vi "DependencyInspector.vi"(11 "Command Line Args":string[](array[string])) -> (0 "error out":errorcluster)   [LabVIEW 2020]
uses:
  UserInterface/UIManager/UIManager.lvclass
  DependencyInspection/CDependencyInspector/CDependencyInspection.lvclass
  d0761231-40dd-4f31-a9c2-62fc8e3657c5.vi/7b12b900-cc26-46dd-9914-f7ad3c9b8ec3.vi
  d0761231-40dd-4f31-a9c2-62fc8e3657c5.vi/1ae99417-134e-4b73-ab04-c2e7cd0032f4.vi
  1cd16c6c-eb87-41a4-aacc-b8daba8fd5f3.vi/7b12b900-cc26-46dd-9914-f7ad3c9b8ec3.vi
  1cd16c6c-eb87-41a4-aacc-b8daba8fd5f3.vi/1ae99417-134e-4b73-ab04-c2e7cd0032f4.vi
  <vilib>/Utility/LVClass/Get LV Class Default Value.vi
panel:
  out "Error Log":string
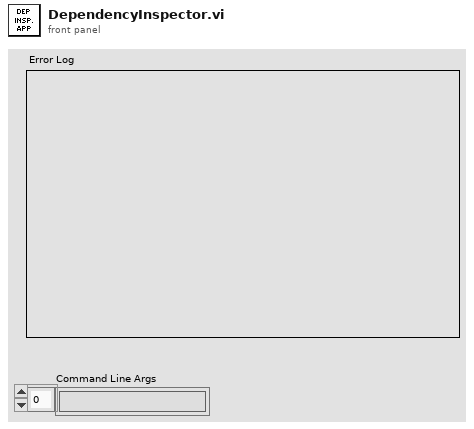
[diagram p1: front panel]
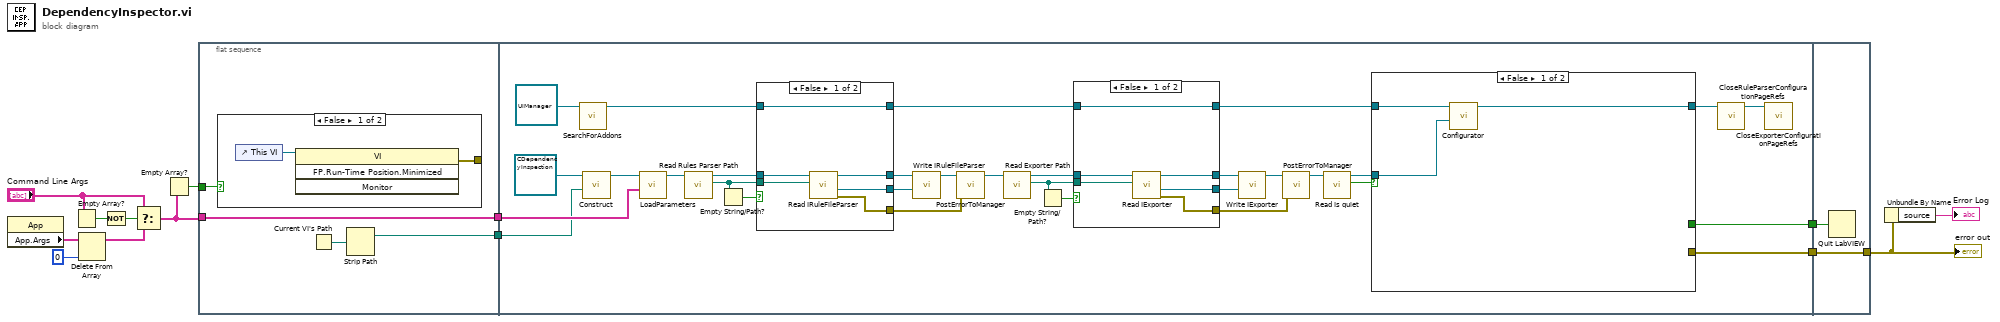
[diagram p0: block diagram]
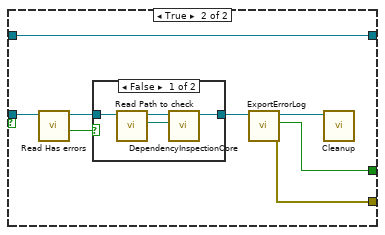
[diagram p3: hidden frame]
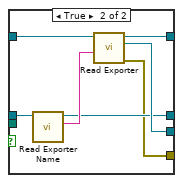
[diagram p5: hidden frame]
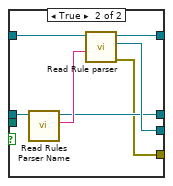
[diagram p6: hidden frame]
diagram:
  n1 = property class="App"() -> ("App.Args"=w11:string[])  [unwired: 2 in, 2 out]
  n2 = Empty Array?(array="Command Line Args") -> (empty?=w5:bool)
  n3 = Delete From Array(array=w11, index=0) -> (array with subset deleted=w4:string[])  [unwired: 1 in, 1 out]
  n4 = Not(x=w5) -> (.not. x?=w1:bool)
  n5 = Select(t="Command Line Args", s=w1, f=w4) -> (s? t:f=w3:string[])
  n6 = Empty Array?(array=w3) -> (empty?=w12:bool)
  n7 = flat-sequence {
    tunnel: w3 -> [w18]
    tunnel: [w18] -> w13
    tunnel: w12 -> [w17]
    tunnel: [w15] -> w10
    tunnel: w13 -> [w33]
    tunnel: w10 -> [w28]
    tunnel: [w32] -> w9
    tunnel: [w31] -> w8
    tunnel: [w95] -> w7
    tunnel: w9 -> [w95]
    tunnel: w8 -> [w94]
    frame #0 {
      n8 = case shown="False" w17 {
        tunnel: [w19 _] -> _
        frame False {
          n9 = control-ref of="This VI"() -> (w20:refnum<vi>)
          n10 = invoke class="VI" method="FP.Run-Time Position.Minimized"(reference=w20) -> (error out=w19:errorcluster)  [unwired: 3 in, 3 out]
        }
        frame True {
        }
      }
      n11 = Current VI's Path() -> (path=w16:path)
      n12 = Strip Path(path=w16) -> (stripped path=w15:path)  [unwired: 1 out]
    }
    frame #1 {
      n13 = call-dynamic "SearchForAddons.vi"("UIManager in"=refnum<class "UIManager.lvclass"> refnum) -> ("UIManager out"=w50:refnum<class "UIManager.lvclass">)  [unwired: 9 in, 1 out]
      n14 = call-dynamic "Construct.vi"("App path"=w28, "CDependencyInspector in"=refnum<class "CDependencyInspection.lvclass"> refnum) -> ("CDependencyInspector out"=w35:refnum<class "CDependencyInspection.lvclass">)  [unwired: 8 in, 1 out]
      n15 = call-dynamic "LoadParameters.vi"("Command line args"=w33, "CDependencyInspection in"=w35) -> ("CDependencyInspection out"=w21:refnum<class "CDependencyInspection.lvclass">)  [unwired: 8 in, 1 out]
      n16 = call-dynamic "Read Rules Parser Path.vi"("CDependencyInspection in"=w21) -> ("Path"=w41:path, "CDependencyInspection out"=w46:refnum<class "CDependencyInspection.lvclass">)  [unwired: 9 in]
      n17 = Empty String/Path?(string/path=w41) -> (empty?=w45:bool)
      n18 = case shown="False" w45 {
        tunnel: w50 -> [w86 w93]
        tunnel: [w86 w92] -> w49
        tunnel: [w84 w88] -> w43
        tunnel: w46 -> [w85 w90]
        tunnel: [w82 w89] -> w42
        tunnel: w41 -> [w83 _]
        tunnel: [w81 w87] -> w25
        frame False {
          n19 = call-dynamic "Read IRuleFileParser.vi"("Path"=w83, "CDependencyInspection in"=w85) -> ("error out"=w81:errorcluster, "IRuleFileParser"=w82:refnum<class "IRuleFileParser.lvclass">, "CDependencyInspection out"=w84:refnum<class "CDependencyInspection.lvclass">)  [unwired: 7 in]
        }
        frame True {
          n20 = call-dynamic "Read Rules Parser Name.vi"("CDependencyInspection in"=w90) -> ("Name"=w91:string, "CDependencyInspection out"=w88:refnum<class "CDependencyInspection.lvclass">)  [unwired: 9 in]
          n21 = call-dynamic "Read Rule parser.vi"("Selection"=w91, "UIManager in"=w93) -> ("error out"=w87:errorcluster, "IRuleFileParser.lvclass"=w89:refnum<class "IRuleFileParser.lvclass">, "UIManager out"=w92:refnum<class "UIManager.lvclass">)  [unwired: 5 in, 2 out]
        }
      }
      n22 = call-dynamic "Write IRuleFileParser.vi"("IRuleFileParser"=w42, "CDependencyInspection in"=w43) -> ("CDependencyInspection out"=w27:refnum<class "CDependencyInspection.lvclass">)  [unwired: 9 in]
      n23 = call-dynamic "PostErrorToManager.vi"("error in (no error)"=w25, "CDependencyInspection in"=w27) -> ("CDependencyInspection out"=w26:refnum<class "CDependencyInspection.lvclass">)  [unwired: 8 in, 1 out]
      n24 = call-dynamic "Read Exporter Path.vi"("CDependencyInspection in"=w26) -> ("Path"=w38:path, "CDependencyInspection out"=w47:refnum<class "CDependencyInspection.lvclass">)  [unwired: 9 in]
      n25 = Empty String/Path?(string/path=w38) -> (empty?=w44:bool)
      n26 = case shown="False" w44 {
        tunnel: w49 -> [w73 w80]
        tunnel: [w73 w79] -> w48
        tunnel: [w71 w75] -> w40
        tunnel: w47 -> [w72 w77]
        tunnel: [w70 w76] -> w39
        tunnel: w38 -> [w69 _]
        tunnel: [w68 w74] -> w22
        frame False {
          n27 = call-dynamic "Read IExporter.vi"("Path"=w69, "CDependencyInspection in"=w72) -> ("error out"=w68:errorcluster, "IExporter"=w70:refnum<class "IExporter.lvclass">, "CDependencyInspection out"=w71:refnum<class "CDependencyInspection.lvclass">)  [unwired: 7 in]
        }
        frame True {
          n28 = call-dynamic "Read Exporter Name.vi"("CDependencyInspection in"=w77) -> ("Name"=w78:string, "CDependencyInspection out"=w75:refnum<class "CDependencyInspection.lvclass">)  [unwired: 9 in]
          n29 = call-dynamic "Read Exporter.vi"("Selection"=w78, "UIManager in"=w80) -> ("error out"=w74:errorcluster, "IExporter.lvclass"=w76:refnum<class "IExporter.lvclass">, "UIManager out"=w79:refnum<class "UIManager.lvclass">)  [unwired: 5 in, 2 out]
        }
      }
      n30 = call-dynamic "Write IExporter.vi"("IExporter"=w39, "CDependencyInspection in"=w40) -> ("CDependencyInspection out"=w24:refnum<class "CDependencyInspection.lvclass">)  [unwired: 9 in]
      n31 = call-dynamic "PostErrorToManager.vi"("error in (no error)"=w22, "CDependencyInspection in"=w24) -> ("CDependencyInspection out"=w23:refnum<class "CDependencyInspection.lvclass">)  [unwired: 8 in, 1 out]
      n32 = call-dynamic "Read Is quiet.vi"("CDependencyInspection in"=w23) -> ("quiet?"=w34:bool, "CDependencyInspection out"=w37:refnum<class "CDependencyInspection.lvclass">)  [unwired: 9 in]
      n33 = case shown="False" w34 {
        tunnel: w48 -> [w54 w62]
        tunnel: w37 -> [w53 w56]
        tunnel: [_ w58] -> w31
        tunnel: [_ w59] -> w32
        tunnel: [w52 w62] -> w29
        frame False {
          n34 = call-dynamic "Configurator.vi"("CDependencyInspector in"=w53, "UIManager in"=w54) -> ("UIManager out"=w52:refnum<class "UIManager.lvclass">)  [unwired: 9 in]
        }
        frame True {
          n35 = call-dynamic "Read Has errors.vi"("CDependencyInspection in"=w56) -> ("empty?"=w55:bool, "CDependencyInspection out"=w57:refnum<class "CDependencyInspection.lvclass">)  [unwired: 9 in]
          n36 = case shown="False" w55 {
            tunnel: w57 -> [w66 w67]
            tunnel: [w65 w67] -> w61
            frame False {
              n37 = call-dynamic "Read Path to check.vi"("CDependencyInspection in"=w66) -> ("Path to check"=w63:path, "CDependencyInspection out"=w64:refnum<class "CDependencyInspection.lvclass">)  [unwired: 9 in]
              n38 = call-dynamic "DependencyInspectionCore.vi"("Path to Check"=w63, "CDependencyInspection in"=w64) -> ("CDependencyInspection out"=w65:refnum<class "CDependencyInspection.lvclass">)  [unwired: 9 in]
            }
            frame True {
            }
          }
          n39 = call-dynamic "ExportErrorLog.vi"("CDependencyInspection in"=w61) -> ("error out"=w59:errorcluster, "Succeeded?"=w58:bool, "CDependencyInspection out"=w60:refnum<class "CDependencyInspection.lvclass">)  [unwired: 8 in]
          n40 = call-dynamic "Cleanup.vi"("CDependencyInspection in"=w60) -> ()  [unwired: 9 in, 2 out]
        }
      }
      n41 = call "CloseRuleParserConfigurationPageRefs.vi"("UIManager in"=w29) -> ("UIManager out"=w30:refnum<class "UIManager.lvclass">)  [unwired: 9 in, 1 out]
      n42 = call "CloseExporterConfigurationPageRefs.vi"("UIManager in"=w30) -> ()  [unwired: 9 in, 2 out]
    }
    frame #2 {
      n43 = Quit LabVIEW(quit? (T)=w94) -> ()
    }
  }
  n44 = Unbundle By Name(w7) -> ("source"=→"Error Log":string)
  "error out" <- w7
